vi "HOST.vi"() -> ()   [LabVIEW 2018]
uses:
  <vilib>/userdefined/High Color/nirio_resource_hc.ctl
  <instrlib>/niDCPower/nidcpower.llb/niDCPower Measurement Type.ctl
  <vilib>/FPGAPlugInAG/PXI-7953R/niLvFpga_Open_PXI-7953R.vi
  <vilib>/rvi/interface/common/dynamic/niFpgaDynamicAddResources.vi
  <vilib>/FPGAPlugInAG/Dynamic/niLvFpga_Reset_Dynamic.vi
  <vilib>/FPGAPlugInAG/Dynamic/niLvFpga_Run_Dynamic.vi
  <vilib>/Utility/error.llb/Error Cluster From Error Code.vi
  <vilib>/rvi/errors/niLvFpgaAdjustHostInterfaceError.vi
  <vilib>/FPGAPlugInAG/Dynamic/niLvFpga_Close_Dynamic.vi
  <vilib>/rvi/interface/nirviOpenFPGA/nirviOpenFPGA.xnode
  FPGA Bitfiles/GSENSE2020_FPGATarget_Target_dmqGfihq6bQ.lvbitx
  <vilib>/rvi/interface/nirviMethod/nirviMethod.xnode
  <vilib>/rvi/interface/nirviReadWriteControl/nirviReadWriteControl.xnode
  <vilib>/rvi/interface/nirviCloseFPGA/nirviCloseFPGA.xnode
  <vilib>/rvi/errors/niLvFpgaMergeErrorWithErrorCode.vi
  <vilib>/rvi/interface/Simulation/niFpgaSimulationCallBeginRW.vi
  <vilib>/FPGAPlugInAG/Dynamic/niLvFpga_ReadFifo_Dynamic.vi
  NiFpgaLv.dll
panel:
  in  "Коррекция":i32
  in  "SYNC":bool
  out "Temp":u16
  out "SEU":bool
  out "Записали адресов":u32
  out "SEU":u16
  out "REG":bool
  out "SEL":bool
  in  "Проверка \n   сбоев":bool
  in  "resource name 2":T1="PXI1Slot9"
  out "SPI_OUT":bool[](array[boolean])
  in  "W(T)/R(F)":bool=TRUE
  in  "Запись":bool[](array[boolean])=[TRUE, TRUE, FALSE, FALSE, FALSE, FALSE, FALSE, FALSE, TRUE, FALSE, TRUE, FALSE, TRUE, TRUE, TRUE, FALSE, FALSE, TRUE, FALSE, FALSE, TRUE, TRUE, FALSE, FALSE, TRUE, TRUE, FALSE, TRUE, TRUE, TRUE, FALSE, FALSE, FALSE, TRUE, TRUE, FALSE, FALSE, TRUE, TRUE, TRUE, TRUE, FALSE, FALSE, TRUE, FALSE, TRUE, FALSE, FALSE, FALSE, TRUE, FALSE, TRUE, TRUE, FALSE, TRUE, TRUE, TRUE, TRUE, TRUE, FALSE, TRUE, TRUE, TRUE, FALSE, TRUE, FALSE, FALSE, FALSE, TRUE, TRUE, TRUE, FALSE, FALSE, FALSE, FALSE, FALSE, FALSE, FALSE, FALSE, FALSE, FALSE, FALSE, FALSE, FALSE, FALSE, FALSE, TRUE, TRUE, TRUE, TRUE, FALSE, FALSE, FALSE, FALSE, FALSE, TRUE, TRUE, FALSE, TRUE, FALSE, TRUE, FALSE, FALSE, FALSE, FALSE, TRUE, FALSE, FALSE, FALSE, TRUE, TRUE, FALSE, TRUE, FALSE, FALSE, FALSE, TRUE, TRUE, TRUE, TRUE, TRUE, FALSE, FALSE, TRUE, FALSE, FALSE, FALSE, TRUE, TRUE, FALSE, TRUE, FALSE, FALSE, TRUE, TRUE, TRUE, TRUE, TRUE, TRUE, FALSE, FALSE, TRUE, TRUE, FALSE, FALSE, TRUE, TRUE, TRUE, TRUE, FALSE, FALSE, TRUE, TRUE, FALSE, FALSE, FALSE, FALSE, FALSE, TRUE, TRUE, FALSE, FALSE, TRUE, FALSE, FALSE, FALSE, FALSE, FALSE, FALSE, FALSE, FALSE, FALSE, FALSE, FALSE, FALSE, FALSE, FALSE, FALSE, FALSE, FALSE, TRUE, FALSE, FALSE, FALSE, FALSE, FALSE, FALSE, FALSE, TRUE, TRUE, FALSE, TRUE, TRUE, TRUE, TRUE, FALSE, TRUE, FALSE, FALSE, FALSE, FALSE, FALSE, FALSE, FALSE, FALSE, FALSE, FALSE, TRUE, TRUE, TRUE, TRUE, TRUE, TRUE, TRUE, TRUE, FALSE, FALSE, TRUE, TRUE, FALSE, FALSE, TRUE, TRUE, TRUE, TRUE, TRUE, TRUE, TRUE, FALSE, FALSE, FALSE, FALSE, TRUE, TRUE, TRUE, FALSE, TRUE, TRUE, FALSE, TRUE, FALSE, TRUE, FALSE, FALSE, FALSE, FALSE, FALSE, FALSE, FALSE, TRUE, TRUE, TRUE, FALSE, TRUE, TRUE, FALSE]
  in  "Top(T)/Bot(F)":bool=TRUE
  in  "SPI":bool
  in  "SEU":path=path "C:/VPL/LabView/GSENSE2020BSI/SEU"
  in  "Автомат":bool
  in  "SYS_RESET":bool
  in  "Хватит ждать!":bool
  in  "SEL_Time, ms":u32=100
  out "Номер образца":string="1"
  in  "Светлый (T)\nТемный (F)":bool
  in  "Frames":path=path "C:/VPL/LabView/GSENSE2020BSI/Frames"
  in  "ПРИМЕЧАНИЕ":string
  in  "SAVE":bool
  in  "122880":u32=122880
  in  "FRAME!":bool
  out "Картинка":bool
  out "Image":T2(plugin-control)
  out "Записали FIFO":bool
  in  "For FIFO (56)":i32=56
  in  "MOVIE":bool
  in  "SIM_SEL":bool
  out "VDD35":bool
  out "VDD20":bool
  out "3,3":bool
  out "LDC":bool
  out "VRH":bool
  in  "VDD35_selcur":dbl=0.25 caption="current limit" format="%_6p"
  in  "VDD20_selcur":dbl=0.4 caption="current limit" format="%_6p"
  in  "3,3_selcur":dbl=0.175 caption="current limit" format="%_6p"
  in  "LDC_selcur":dbl=0.01 caption="current limit" format="%_6p"
  in  "VRH_selcur":dbl=0.03 caption="current limit" format="%_6p"
  out "VDD35":u16
  out "VDD20":u16
  out "3,3":u16
  out "LDC":u16
  out "VRH":u16
  in  "Питание":bool
  in  "Стоп":bool
  in  "VDD35, V":dbl=3.51 caption="voltage level" format="%_6p"
  in  "3,3, V":dbl=3.3099999999999996 caption="voltage level" format="%_6p"
  in  "LDC, V":dbl=0.81 caption="voltage level" format="%_6p"
  in  "VRH, V":dbl=3.8099999999999996 caption="voltage level" format="%_6p"
  in  "VDD35_curlim":dbl=0.3 caption="current limit" format="%_6p"
  in  "VDD20_curlim":dbl=0.5 caption="current limit" format="%_6p"
  in  "3,3_curlim":dbl=0.2 caption="current limit" format="%_6p"
  in  "LDC_curlim":dbl=0.015 caption="current limit" format="%_6p"
  in  "LED_curlim":dbl=0.1 caption="current limit" format="%_6p"
  in  "VRH_curlim":dbl=0.05 caption="current limit" format="%_6p"
  out "VDD35_cur":dbl caption="measurement" format="%_6g"
  out "VDD20_cur":dbl caption="measurement" format="%_6g"
  out "3,3_cur":dbl caption="measurement" format="%_6g"
  out "LDC_cur":dbl caption="measurement" format="%_6g"
  out "LED_cur":dbl caption="measurement" format="%_6g"
  out "VRH_cur":dbl caption="measurement" format="%_6g"
  in  "VDD20, V":dbl=2.01 caption="voltage level" format="%_6p"
  in  "LED, V":dbl=6.0 caption="voltage level" format="%_6p"
  out "VDD35_char":dbl(graph)=-0.007753012065680951
  out "VDD20_char":dbl(graph)=6.909391540672134e-05
  out "3,3_char":dbl(graph)=9.424895165128459e-05
  out "LDC_char":dbl(graph)=-9.950040532110056e-06
  out "LED_char":dbl(graph)=9.067752968783287e-05
  out "VRH_char":dbl(graph)=1.5967060684808935e-06
  in  "LED":bool caption="output enabled"
  in  "0":refnum<k15>="PXI1Slot5" caption="1"
  in  "1":refnum<k15>="PXI1Slot6"
  in  "2":refnum<k15>="PXI1Slot7" caption="1"
  in  "SEL":path=path "C:/VPL/LabView/GSENSE2020BSI/SEL"
  out "Data":u8[][](array[numeric])
  out "Array":u32[][](array[numeric])
  # "Bot_ch - HIGH gain"
  # "Прибавка 124 сбоев связана с ТЭ"
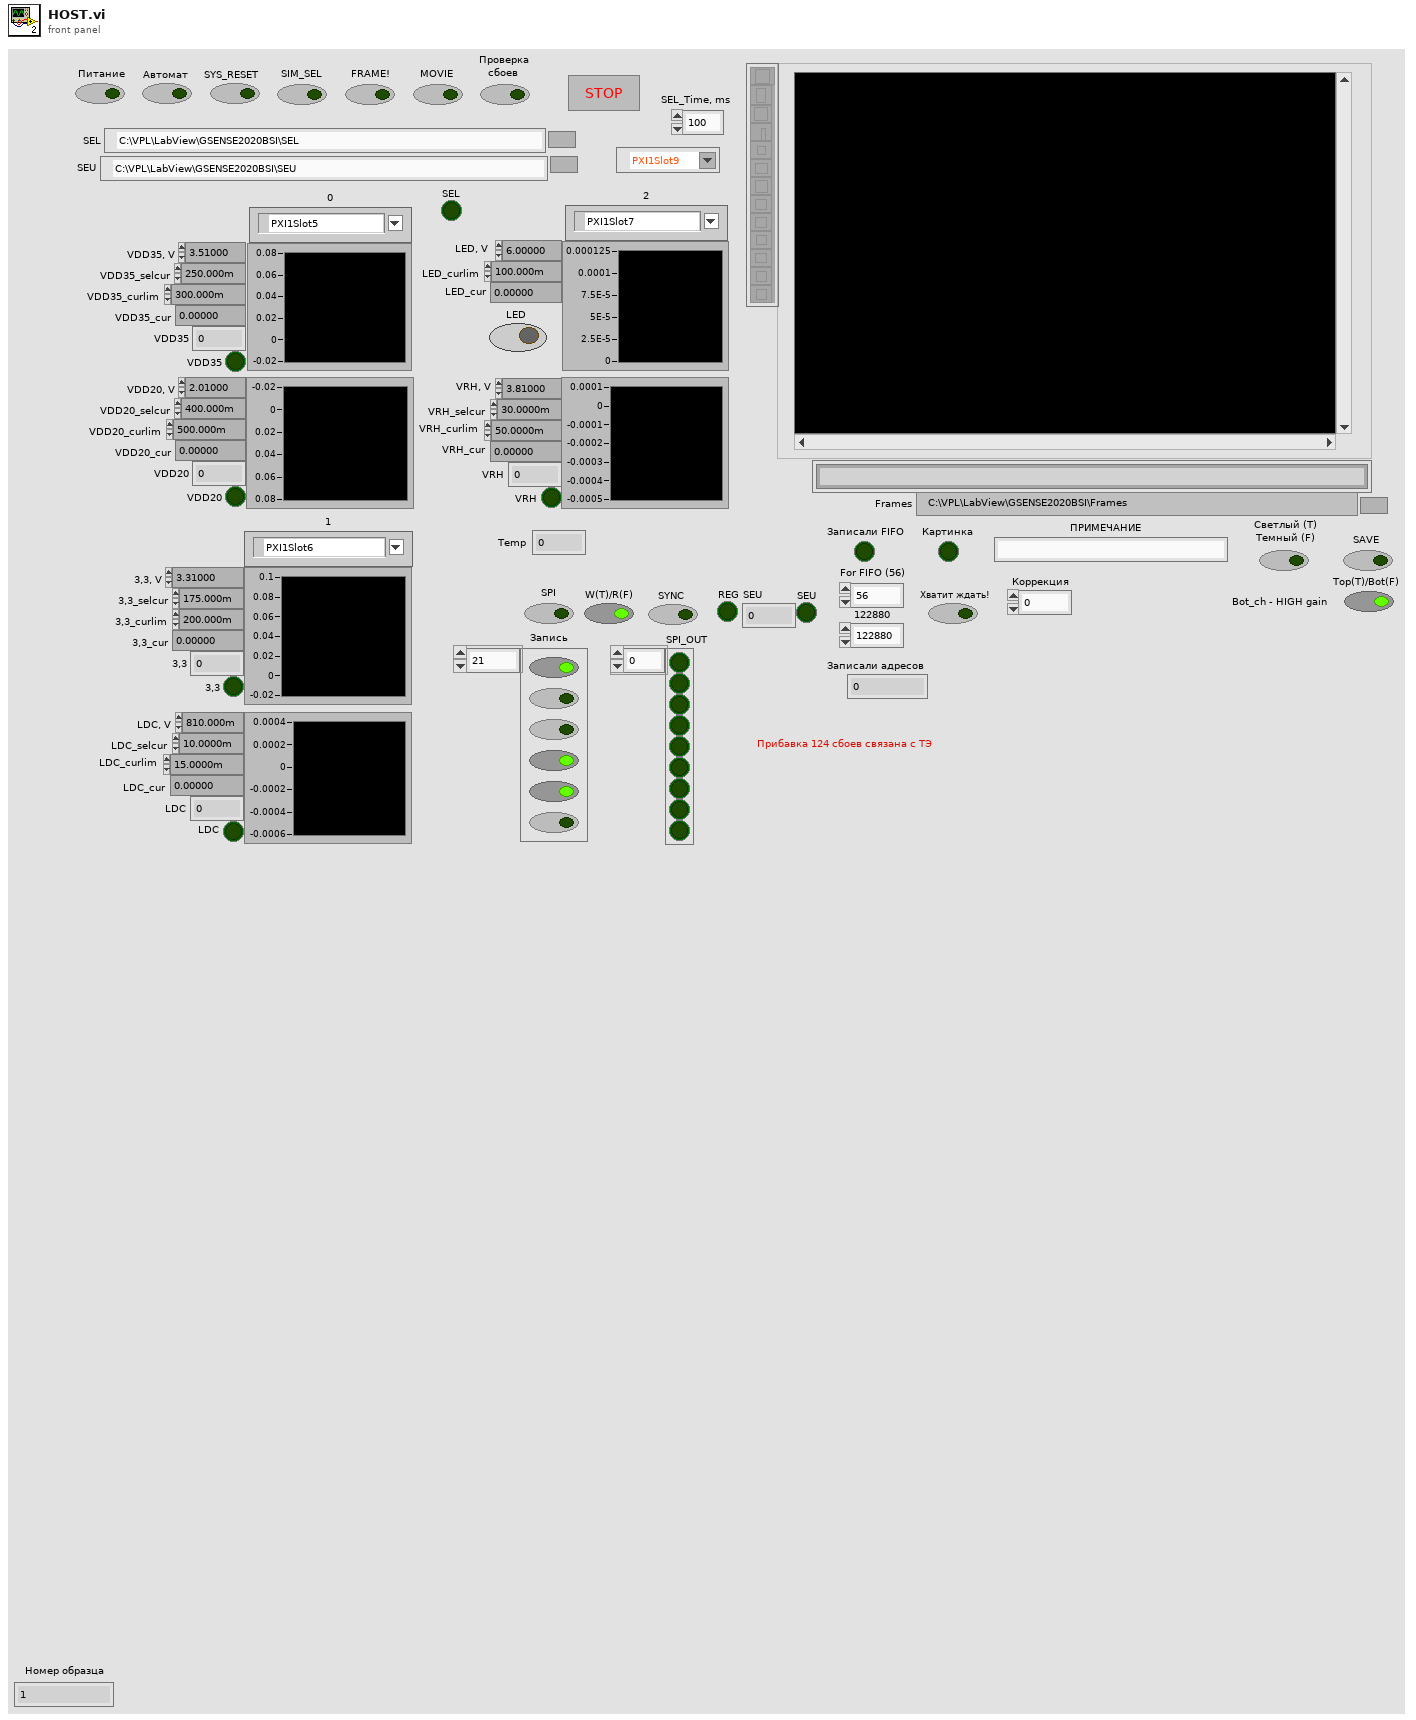
[diagram p1: front panel]
types:
  T1 = typedef "nirio_resource_hc.ctl" = tag
  T2 = typedef "IMAQ Image.ctl" = refnum<image>
  T3 = typedef "Image Type" = u32
  T4 = enum16{"open", "replace", "create", "open or create", "replace or create", "replace or create with confirmation"}
  T5 = typedef "niDCPower Measurement Type.ctl" = i32
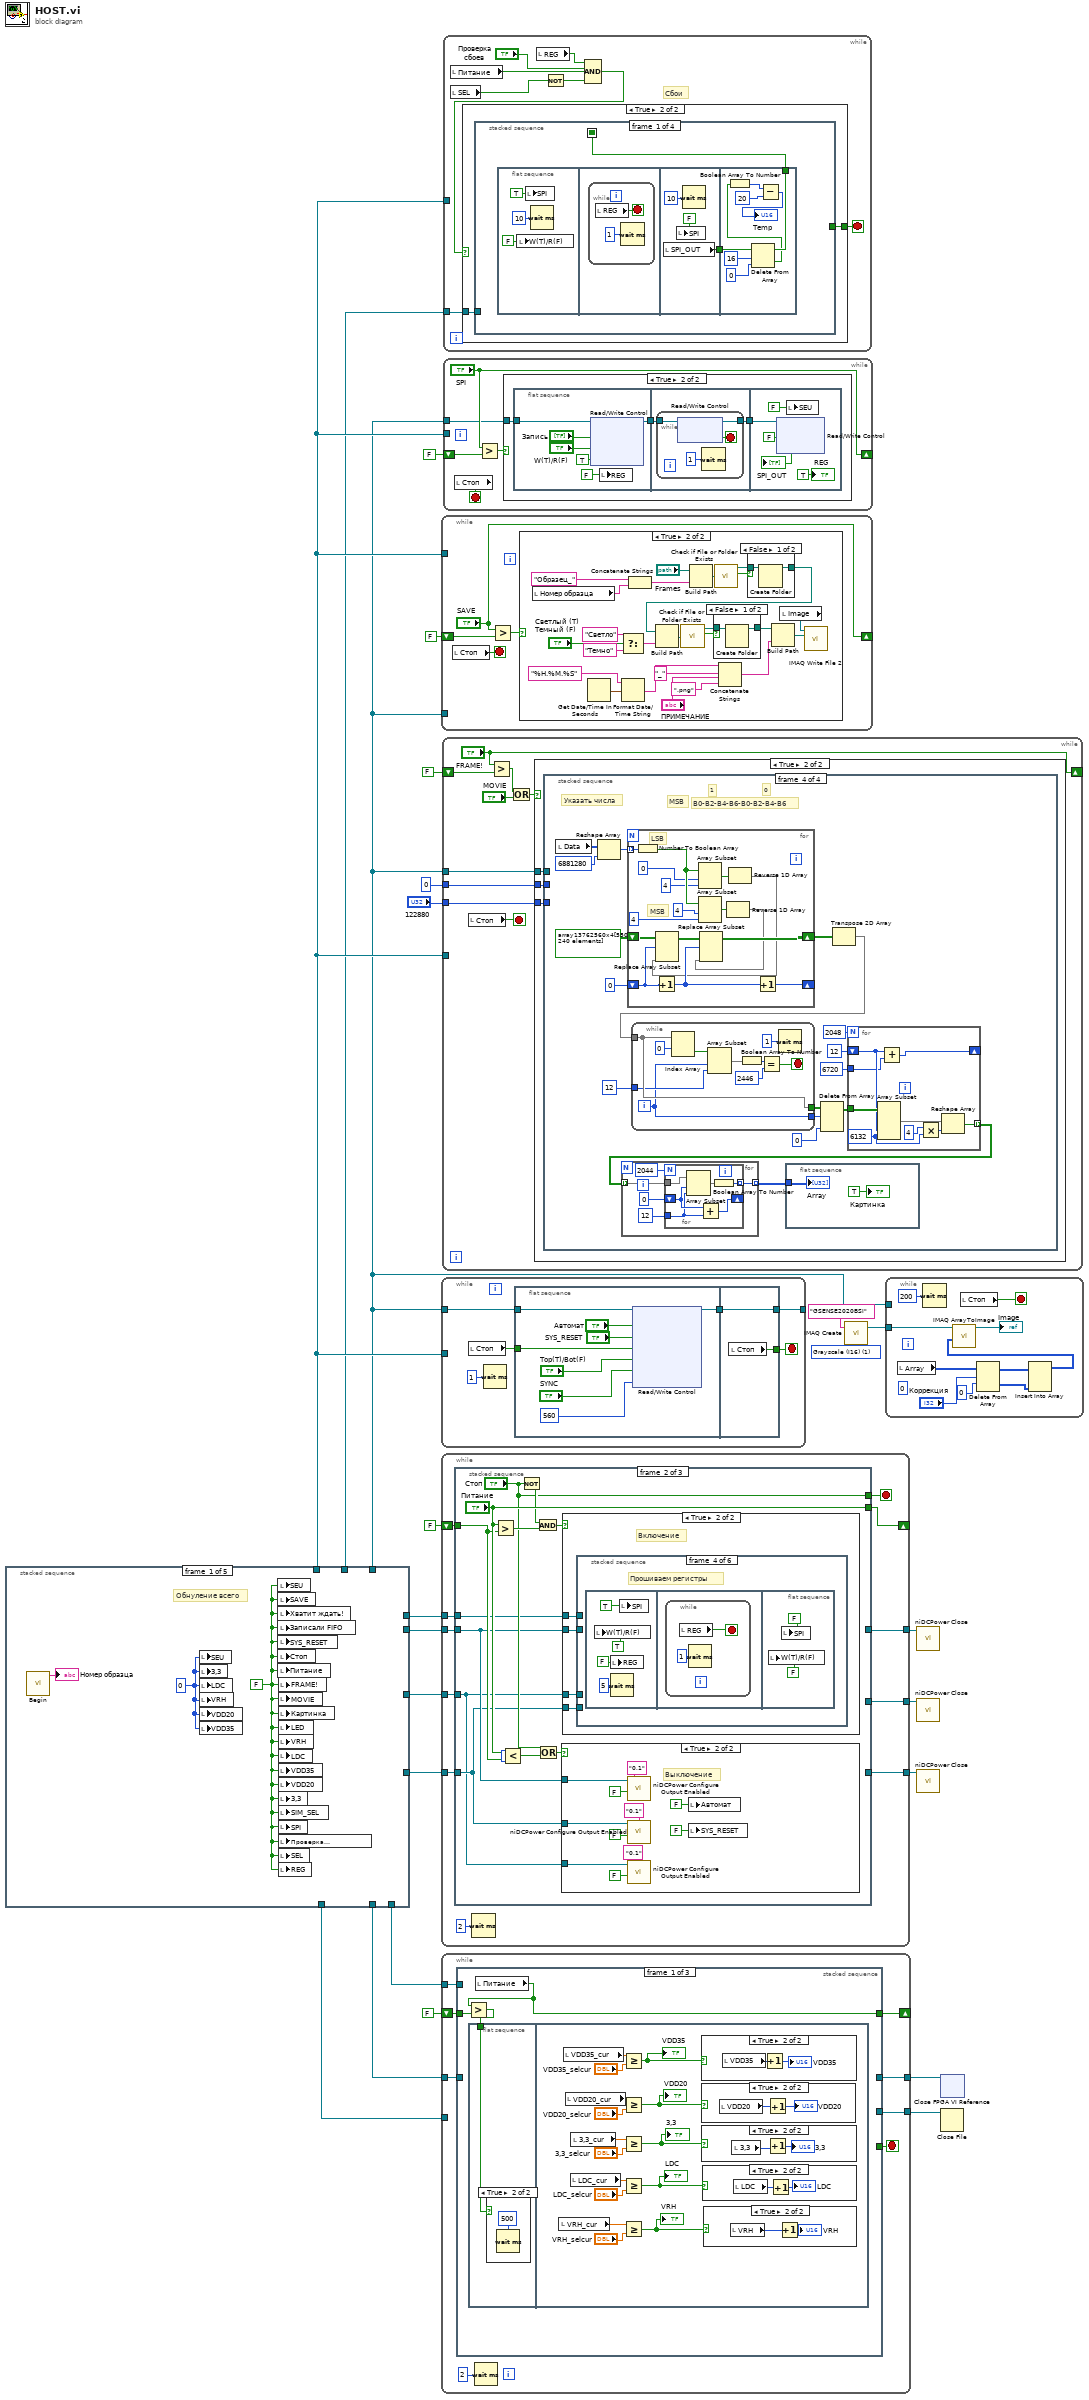
[diagram p0: block diagram]
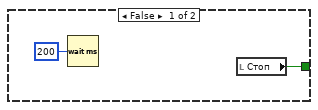
[diagram p2: hidden frame]
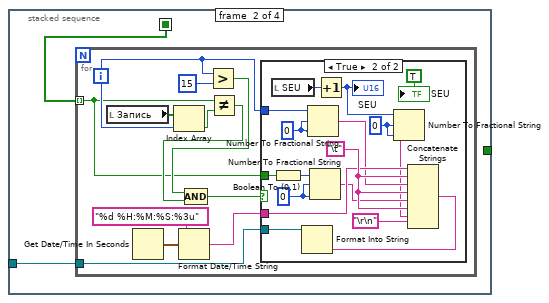
[diagram p3: hidden frame]
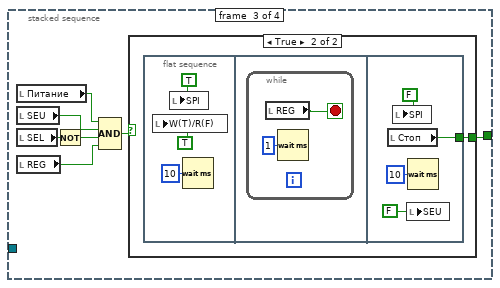
[diagram p5: hidden frame]
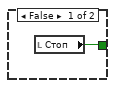
[diagram p6: hidden frame]
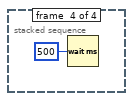
[diagram p7: hidden frame]
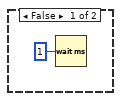
[diagram p8: hidden frame]
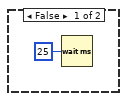
[diagram p9: hidden frame]
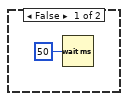
[diagram p12: hidden frame]
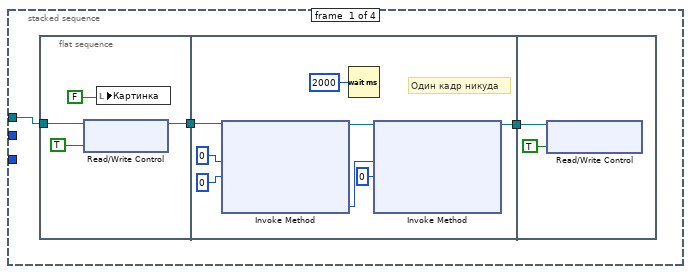
[diagram p13: hidden frame]
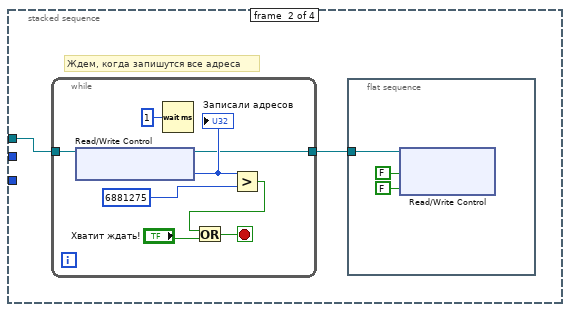
[diagram p14: hidden frame]
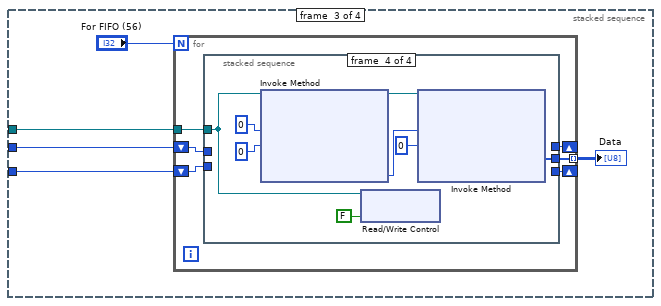
[diagram p15: hidden frame]
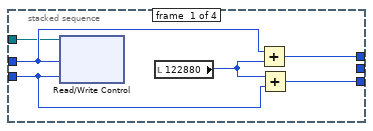
[diagram p16: hidden frame]
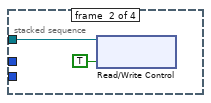
[diagram p17: hidden frame]
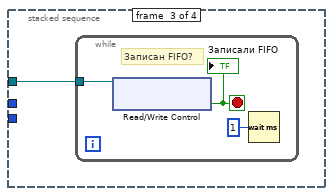
[diagram p18: hidden frame]
diagram:
  w3 = T3 1 items=["Grayscale (U8)", "Grayscale (I16)", "Grayscale (SGL)", "Complex (CSG)", "RGB (U32)", "HSL (U32)", "RGB (U64)"] ("Image Type")
  n1 = stacked-sequence {
    tunnel: [_ _ _ _ w103] -> w23
    tunnel: [_ _ _ _ w104] -> w25
    tunnel: [_ _ _ _ w108] -> w24
    tunnel: [_ _ _ w100 _] -> w1
    tunnel: [_ _ _ w100 _] -> w17
    tunnel: [_ w37 _ _ _] -> w18
    tunnel: [_ _ _ _ w104] -> w9
    tunnel: [_ _ _ _ w103] -> w12
    tunnel: [_ _ w67 _ _] -> w5
    tunnel: [_ _ _ w100 _] -> w6
    frame #0 {
      w26 = FALSE ("Стоп")
      w27 = u16 0 ("ADC")
      # "Обнуление всего"
      n2 = call "Begin.vi"() -> ("Номер образца 2"=→"Номер образца":string)  [unwired: 11 in]
      n3 = local write "SEU"(w27) -> ()
      n4 = local write "3,3"(w27) -> ()
      n5 = local write "LDC"(w27) -> ()
      n6 = local write "VRH"(w27) -> ()
      n7 = local write "VDD20"(w27) -> ()
      n8 = local write "VDD35"(w27) -> ()
      n9 = local write "SEU"(w26) -> ()
      n10 = local write "SAVE"(w26) -> ()
      n11 = local write "Хватит ждать!"(w26) -> ()
      n12 = local write "Записали FIFO"(w26) -> ()
      n13 = local write "SYS_RESET"(w26) -> ()
      n14 = local write "Стоп"(w26) -> ()
      n15 = local write "Питание"(w26) -> ()
      n16 = local write "FRAME!"(w26) -> ()
      n17 = local write "MOVIE"(w26) -> ()
      n18 = local write "Картинка"(w26) -> ()
      n19 = local write "LED"(w26) -> ()
      n20 = local write "VRH"(w26) -> ()
      n21 = local write "LDC"(w26) -> ()
      n22 = local write "VDD35"(w26) -> ()
      n23 = local write "VDD20"(w26) -> ()
      n24 = local write "3,3"(w26) -> ()
      n25 = local write "SIM_SEL"(w26) -> ()
      n26 = local write "SPI"(w26) -> ()
      n27 = local write "Проверка \n   сбоев"(w26) -> ()
      n28 = local write "SEL"(w26) -> ()
      n29 = local write "REG"(w26) -> ()
    }
    frame #1 {
      w31 = "\t"
      # "Лог по токам"
      n30 = local read "Номер образца"() -> (w59:string)
      n31 = Build Path(base path="SEL", name or relative path=w59) -> (appended path=w56:path)
      n32 = Get Date/Time In Seconds() -> (seconds since 1Jan1904=w53:timestamp)
      n33 = call <vilib>:"Check if File or Folder Exists.vi"("path"=w56) -> ("file or folder exists?"=w57:bool, "dup path"=w58:path)  [unwired: 8 in, 1 out]
      n34 = Format Date/Time String(time format string (%c)="%d %H.%M.%S", seconds (now)=w53) -> (date/time string=w51:string)  [unwired: 1 in]
      n35 = case shown="False" w57 {
        tunnel: w58 -> [w65 w66]
        tunnel: [w64 w66] -> w29
        frame False {
          n36 = Create Folder(path (use dialog)=w65) -> (created path=w64:path)  [unwired: 2 in, 2 out]
        }
        frame True {
        }
      }
      n37 = Concatenate Strings(w51, ".xls" ("string")) -> (w50:string)
      n38 = Build Path(base path=w29, name or relative path=w50) -> (appended path=w52:path)
      n39 = Open/Create/Replace File(file path (use dialog)=w52, operation (0:open)=T4."open or create", access (0:read/write)=enum16{"read/write", "read-only", "write-only"}."read/write") -> (refnum out=w54:refnum<file>)  [unwired: 3 in, 2 out]
      n40 = case shown="True" TRUE {
        tunnel: w54 -> [w60 w63]
        tunnel: [w60 w61] -> w49
        frame False {
        }
        frame True {
          n41 = Set File Position(refnum=w63, from (0:start)=enum16{"start", "end", "current"}."end") -> (refnum out=w61:refnum<file>)  [unwired: 2 in, 1 out]
        }
      }
      n42 = Format Into String(initial string=w49, "Time" ("input 1"), w31, "VDD35_cur", w31, "VDD20_cur", w31, "3,3_cur", w31, "LDC_cur", w31, "VRH_cur", w31, "VDD35_cur", w31, "VDD20_cur", w31, "3,3_cur", w31, "LDC_cur", w31, "VRH_cur", w31, "\r\n") -> (resulting string=w37:refnum<file>)  [unwired: 2 in, 1 out]
    }
    frame #2 {
      w70 = "\t"
      # "Лог по сбоям"
      n43 = local read "Номер образца"() -> (w74:string)
      n44 = Build Path(base path="SEU", name or relative path=w74) -> (appended path=w88:path)
      n45 = Get Date/Time In Seconds() -> (seconds since 1Jan1904=w86:timestamp)
      n46 = call <vilib>:"Check if File or Folder Exists.vi"("path"=w88) -> ("file or folder exists?"=w89:bool, "dup path"=w90:path)  [unwired: 8 in, 1 out]
      n47 = Format Date/Time String(time format string (%c)="%d %H.%M.%S", seconds (now)=w86) -> (date/time string=w84:string)  [unwired: 1 in]
      n48 = case shown="False" w89 {
        tunnel: w90 -> [w96 w97]
        tunnel: [w95 w97] -> w75
        frame False {
          n49 = Create Folder(path (use dialog)=w96) -> (created path=w95:path)  [unwired: 2 in, 2 out]
        }
        frame True {
        }
      }
      n50 = Concatenate Strings(w84, ".xls" ("string")) -> (w83:string)
      n51 = Build Path(base path=w75, name or relative path=w83) -> (appended path=w85:path)
      n52 = Open/Create/Replace File(file path (use dialog)=w85, operation (0:open)=T4."open or create", access (0:read/write)=enum16{"read/write", "read-only", "write-only"}."read/write") -> (refnum out=w87:refnum<file>)  [unwired: 3 in, 2 out]
      n53 = case shown="True" TRUE {
        tunnel: w87 -> [w91 w94]
        tunnel: [w91 w92] -> w82
        frame False {
        }
        frame True {
          n54 = Set File Position(refnum=w94, from (0:start)=enum16{"start", "end", "current"}."end") -> (refnum out=w92:refnum<file>)  [unwired: 2 in, 1 out]
        }
      }
      n55 = Format Into String(initial string=w82, "Time" ("input 1"), w70, "Регистр №" ("input 3"), w70, "Содержание" ("input 4"), w70, "Кол-во сбоев" ("input 7"), "\r\n") -> (resulting string=w67:refnum<file>)  [unwired: 2 in, 1 out]
    }
    frame #3 {
      n56 = xnode "Open FPGA VI Reference"("resource name"="resource name 2") -> ("FPGA VI Reference Out"=w98:refnum<k20>)  [unwired: 1 in, 1 out]
      n57 = xnode "Invoke Method"("FPGA VI Reference In"=w98) -> ("FPGA VI Reference Out"=w102:refnum<k20>, "error out"=w101:errorcluster)  [unwired: 1 in]
      n58 = xnode "Invoke Method"("FPGA VI Reference In"=w102, "error in"=w101) -> ("FPGA VI Reference Out"=w100:refnum<k20>)  [unwired: 1 in, 1 out]
    }
    frame #4 {
      # "Готово"
      n59 = call <instrlib>:"niDCPower Initialize.vi"("resource name"="2") -> ("error out"=w114:errorcluster, "instrument handle out"=w111:refnum<k15>)  [unwired: 3 in, 6 out]
      n60 = call <instrlib>:"niDCPower Initialize.vi"("resource name"="1") -> ("error out"=w112:errorcluster, "instrument handle out"=w109:refnum<k15>)  [unwired: 3 in, 6 out]
      n61 = call <instrlib>:"niDCPower Initialize.vi"("resource name"="0") -> ("error out"=w113:errorcluster, "instrument handle out"=w110:refnum<k15>)  [unwired: 3 in, 6 out]
      n62 = call <instrlib>:"niDCPower Configure Voltage Level.vi"("error in (no error)"=w114, "voltage level"=0.0, "channel name"="0,1", "instrument handle"=w111) -> ("instrument handle out"=w103:refnum<k15>)  [unwired: 6 in, 1 out]
      n63 = call <instrlib>:"niDCPower Configure Voltage Level.vi"("error in (no error)"=w112, "voltage level"=0.0, "channel name"="0,1", "instrument handle"=w109) -> ("instrument handle out"=w108:refnum<k15>)  [unwired: 6 in, 1 out]
      n64 = call <instrlib>:"niDCPower Configure Voltage Level.vi"("error in (no error)"=w113, "voltage level"=0.0, "channel name"="0,1", "instrument handle"=w110) -> ("instrument handle out"=w104:refnum<k15>)  [unwired: 6 in, 1 out]
    }
  }
  n65 = while {
    tunnel: w1 -> [w125]
    tunnel: [w124] -> _
    tunnel: w9 -> [_]
    stop <- w121 stop-if-true
    n66 = local read "Стоп"() -> (w123:bool)
    n67 = Wait (ms)(milliseconds to wait=u32 1) -> ()  [unwired: 1 out]
    n68 = flat-sequence {
      tunnel: w125 -> [w134]
      tunnel: w123 -> [w132]
      tunnel: [w133] -> w122
      tunnel: [w136] -> w124
      tunnel: w122 -> [w136]
      tunnel: [w135] -> w121
      frame #0 {
        n69 = xnode "Read/Write Control"("FPGA VI Reference In"=w134, "Автомат"="Автомат", "SYS_RESET"="SYS_RESET", "Стоп"=w132, "Top(T)/Bot(F)"="Top(T)/Bot(F)", "SYNC"="SYNC", "480"=u16 560) -> ("FPGA VI Reference Out"=w133:refnum<k20>)  [unwired: 1 in, 1 out]
      }
      frame #1 {
        n70 = local read "Стоп"() -> (w135:bool)
      }
    }
  }
  n71 = while {
    tunnel: w25 -> [w146]
    tunnel: w24 -> [w145]
    tunnel: w23 -> [w144]
    shift-right: [w141] -> _
    shift-left: FALSE -> [w142]
    tunnel: [w140] -> w21
    tunnel: [w139] -> w20
    tunnel: [w138] -> w19
    tunnel: w6 -> [w137]
    stop <- w143 stop-if-true
    n72 = stacked-sequence {
      tunnel: w144 -> [w158 w205 w256]
      tunnel: w146 -> [w160 w206 w258]
      tunnel: w145 -> [w159 w204 w257]
      tunnel: [_ "Стоп" _] -> w143
      tunnel: w142 -> [_ w213 _]
      tunnel: [_ "Питание" _] -> w141
      tunnel: [_ _ w258] -> w140
      tunnel: [_ _ w257] -> w139
      tunnel: [_ _ w256] -> w138
      tunnel: w137 -> [_ w203 _]
      frame #0 {
        w148 = T5 0 items=["Current", "Voltage"] ("measurement type")
        n73 = call <instrlib>:"niDCPower Configure Current Limit.vi"("current limit"="VDD35_curlim", "channel name"="0", "instrument handle"=w160) -> ("instrument handle out"=w183:refnum<k15>)  [unwired: 7 in, 1 out]
        n74 = call <instrlib>:"niDCPower Configure Current Limit.vi"("current limit"="VDD20_curlim", "channel name"="1", "instrument handle"=w160) -> ("instrument handle out"=w184:refnum<k15>)  [unwired: 7 in, 1 out]
        n75 = call <instrlib>:"niDCPower Configure Current Limit.vi"("current limit"="3,3_curlim", "channel name"="0", "instrument handle"=w159) -> ("instrument handle out"=w185:refnum<k15>)  [unwired: 7 in, 1 out]
        n76 = call <instrlib>:"niDCPower Configure Current Limit.vi"("current limit"="LDC_curlim", "channel name"="1", "instrument handle"=w159) -> ("instrument handle out"=w186:refnum<k15>)  [unwired: 7 in, 1 out]
        n77 = call <instrlib>:"niDCPower Configure Current Limit.vi"("current limit"="LED_curlim", "channel name"="0", "instrument handle"=w158) -> ("instrument handle out"=w187:refnum<k15>)  [unwired: 7 in, 1 out]
        n78 = call <instrlib>:"niDCPower Configure Current Limit.vi"("current limit"="VRH_curlim", "channel name"="1", "instrument handle"=w158) -> ("instrument handle out"=w188:refnum<k15>)  [unwired: 7 in, 1 out]
        n79 = call <instrlib>:"niDCPower Configure Voltage Level.vi"("voltage level"="VDD35, V", "channel name"="0", "instrument handle"=w183) -> ("instrument handle out"=w166:refnum<k15>)  [unwired: 7 in, 1 out]
        n80 = call <instrlib>:"niDCPower Configure Voltage Level.vi"("voltage level"="VDD20, V", "channel name"="1", "instrument handle"=w184) -> ("instrument handle out"=w165:refnum<k15>)  [unwired: 7 in, 1 out]
        n81 = call <instrlib>:"niDCPower Configure Voltage Level.vi"("voltage level"="3,3, V", "channel name"="0", "instrument handle"=w185) -> ("instrument handle out"=w164:refnum<k15>)  [unwired: 7 in, 1 out]
        n82 = call <instrlib>:"niDCPower Configure Voltage Level.vi"("voltage level"="LDC, V", "channel name"="1", "instrument handle"=w186) -> ("instrument handle out"=w163:refnum<k15>)  [unwired: 7 in, 1 out]
        n83 = call <instrlib>:"niDCPower Configure Voltage Level.vi"("voltage level"="LED, V", "channel name"="0", "instrument handle"=w187) -> ("instrument handle out"=w162:refnum<k15>)  [unwired: 7 in, 1 out]
        n84 = call <instrlib>:"niDCPower Configure Voltage Level.vi"("voltage level"="VRH, V", "channel name"="1", "instrument handle"=w188) -> ("instrument handle out"=w161:refnum<k15>)  [unwired: 7 in, 1 out]
        n85 = call <instrlib>:"niDCPower Measure.vi"("measurement type"=w148, "channel name"="0", "instrument handle"=w166) -> ("measurement"=→"VDD35_cur" →"VDD35_char":dbl)  [unwired: 6 in, 2 out]
        n86 = call <instrlib>:"niDCPower Measure.vi"("measurement type"=w148, "channel name"="1", "instrument handle"=w165) -> ("measurement"=→"VDD20_cur" →"VDD20_char":dbl)  [unwired: 6 in, 2 out]
        n87 = call <instrlib>:"niDCPower Measure.vi"("measurement type"=w148, "channel name"="0", "instrument handle"=w164) -> ("measurement"=→"3,3_cur" →"3,3_char":dbl)  [unwired: 6 in, 2 out]
        n88 = call <instrlib>:"niDCPower Measure.vi"("measurement type"=w148, "channel name"="1", "instrument handle"=w163) -> ("measurement"=→"LDC_cur" →"LDC_char":dbl)  [unwired: 6 in, 2 out]
        n89 = call <instrlib>:"niDCPower Measure.vi"("measurement type"=w148, "channel name"="0", "instrument handle"=w162) -> ("measurement"=→"LED_cur" →"LED_char":dbl, "instrument handle out"=w151:refnum<k15>)  [unwired: 6 in, 1 out]
        n90 = call <instrlib>:"niDCPower Measure.vi"("measurement type"=w148, "channel name"="1", "instrument handle"=w161) -> ("measurement"=→"VRH_cur" →"VRH_char":dbl)  [unwired: 6 in, 2 out]
        n91 = call <instrlib>:"niDCPower Configure Output Enabled.vi"("output enabled"="LED", "channel name"="0", "instrument handle"=w151) -> ()  [unwired: 7 in, 2 out]
      }
      frame #1 {
        n92 = Greater?(x="Питание", y=w213) -> (0:w210:bool)
        n93 = Less?(x="Питание", y=w213) -> (x < y?=w208:bool)
        n94 = Not(x="Стоп") -> (.not. x?=w209:bool)
        n95 = And(x=w209, y=w210) -> (x .and. y?=w212:bool)
        n96 = Or(x="Стоп", y=w208) -> (x .or. y?=w211:bool)
        n97 = case shown="True" w211 {
          tunnel: w206 -> [_ w225]
          tunnel: w205 -> [_ w224]
          tunnel: w204 -> [_ w223]
          frame False {
          }
          frame True {
            # "Выключение"
            n98 = call <instrlib>:"niDCPower Configure Output Enabled.vi"("output enabled"=FALSE, "channel name"="0,1", "instrument handle"=w225) -> ()  [unwired: 7 in, 2 out]
            n99 = call <instrlib>:"niDCPower Configure Output Enabled.vi"("output enabled"=FALSE, "channel name"="0,1", "instrument handle"=w224) -> ()  [unwired: 7 in, 2 out]
            n100 = call <instrlib>:"niDCPower Configure Output Enabled.vi"("output enabled"=FALSE, "channel name"="0,1", "instrument handle"=w223) -> ()  [unwired: 7 in, 2 out]
            n101 = local write "Автомат"(FALSE ("Автомат")) -> ()
            n102 = local write "SYS_RESET"(FALSE ("SYS_RESET")) -> ()
          }
        }
        n103 = case shown="True" w212 {
          tunnel: w206 -> [_ w229]
          tunnel: w204 -> [_ w228]
          tunnel: w205 -> [_ w227]
          tunnel: w203 -> [_ w226]
          frame False {
          }
          frame True {
            # "Включение"
            n104 = stacked-sequence {
              tunnel: w229 -> [w233 _ _ _ _ _]
              tunnel: w228 -> [w232 _ _ _ _ w251]
              tunnel: w227 -> [_ _ _ _ _ w250]
              tunnel: w226 -> [_ _ _ _ _ _]
              frame #0 {
                # "3,3"
                # "VDD20"
                # "VDD35(PIX)"
                n105 = call <instrlib>:"niDCPower Configure Output Enabled.vi"("output enabled"=TRUE, "channel name"="0", "instrument handle"=w233) -> ()  [unwired: 7 in, 2 out]
                n106 = call <instrlib>:"niDCPower Configure Output Enabled.vi"("output enabled"=TRUE, "channel name"="1", "instrument handle"=w233) -> ()  [unwired: 7 in, 2 out]
                n107 = call <instrlib>:"niDCPower Configure Output Enabled.vi"("output enabled"=TRUE, "channel name"="0", "instrument handle"=w232) -> ()  [unwired: 7 in, 2 out]
              }
              frame #1 {
                n108 = Wait (ms)(milliseconds to wait=u32 50) -> ()  [unwired: 1 out]
              }
              frame #2 {
                n109 = local write "Автомат"(TRUE ("Автомат")) -> ()
              }
              frame #3 {
                # "Прошиваем регистры"
                n110 = flat-sequence {
                  frame #0 {
                    n111 = local write "W(T)/R(F)"(TRUE ("W(T)/R(F)")) -> ()
                    n112 = local write "REG"(FALSE ("REG")) -> ()
                    n113 = Wait (ms)(milliseconds to wait=u32 5) -> ()  [unwired: 1 out]
                    n114 = local write "SPI"(TRUE ("SPI")) -> ()
                  }
                  frame #1 {
                    n115 = while {
                      stop <- w244 stop-if-true
                      n116 = local read "REG"() -> (w244:bool)
                      n117 = Wait (ms)(milliseconds to wait=u32 1) -> ()  [unwired: 1 out]
                    }
                  }
                  frame #2 {
                    n118 = local write "W(T)/R(F)"(FALSE ("W(T)/R(F)")) -> ()
                    n119 = local write "SPI"(FALSE ("SPI")) -> ()
                  }
                }
              }
              frame #4 {
                n120 = Wait (ms)(milliseconds to wait=u32 1) -> ()  [unwired: 1 out]
              }
              frame #5 {
                # "VRH"
                # "LDC"
                n121 = call <instrlib>:"niDCPower Configure Output Enabled.vi"("output enabled"=TRUE, "channel name"="1", "instrument handle"=w251) -> ()  [unwired: 7 in, 2 out]
                n122 = call <instrlib>:"niDCPower Configure Output Enabled.vi"("output enabled"=TRUE, "channel name"="1", "instrument handle"=w250) -> ()  [unwired: 7 in, 2 out]
                n123 = local write "SYS_RESET"(TRUE ("SYS_RESET")) -> ()
              }
            }
          }
        }
      }
      frame #2 {
      }
    }
    n124 = Wait (ms)(milliseconds to wait=u32 2) -> ()  [unwired: 1 out]
  }
  n125 = while {
    tunnel: w17 -> [w261]
    shift-right: [w265] -> _
    shift-left: FALSE ("Питание") -> [w266]
    tunnel: w18 -> [w263]
    tunnel: w12 -> [_]
    tunnel: [w260] -> w11
    tunnel: [w259] -> w10
    stop <- w262 stop-if-true
    n126 = stacked-sequence {
      tunnel: w266 -> [w269 _ _]
      tunnel: [w268 _ _] -> w265
      tunnel: w263 -> [_ w330 _]
      tunnel: [_ _ w346] -> w262
      tunnel: w261 -> [_ _ w345]
      tunnel: [_ w297 _] -> w260
      tunnel: [_ _ w336] -> w259
      frame #0 {
        n127 = flat-sequence {
          tunnel: w267 -> [w270]
          frame #0 {
            n128 = case shown="True" w270 {
              frame False {
              }
              frame True {
                n129 = Wait (ms)(milliseconds to wait=u32 500) -> ()  [unwired: 1 out]
              }
            }
          }
          frame #1 {
            n130 = local read "VRH_cur"() -> (w277:dbl)
            n131 = local read "VDD35_cur"() -> (w279:dbl)
            n132 = local read "VDD20_cur"() -> (w280:dbl)
            n133 = local read "LDC_cur"() -> (w282:dbl)
            n134 = local read "3,3_cur"() -> (w281:dbl)
            n135 = Greater Or Equal?(x=w279, y="VDD35_selcur") -> (x >= y?=w276:bool)
            "VDD35" <- w276
            n136 = Greater Or Equal?(x=w280, y="VDD20_selcur") -> (x >= y?=w275:bool)
            "VDD20" <- w275
            n137 = Greater Or Equal?(x=w281, y="3,3_selcur") -> (x >= y?=w274:bool)
            "3,3" <- w274
            n138 = Greater Or Equal?(x=w282, y="LDC_selcur") -> (x >= y?=w273:bool)
            "LDC" <- w273
            n139 = Greater Or Equal?(x=w277, y="VRH_selcur") -> (x >= y?=w272:bool)
            "VRH" <- w272
            n140 = case shown="True" w276 {
              frame False {
              }
              frame True {
                n141 = local read "VDD35"() -> (w295:u16)
                n142 = Increment(x=w295) -> (x+1=→"VDD35":u16)
              }
            }
            n143 = case shown="True" w275 {
              frame False {
              }
              frame True {
                n144 = local read "VDD20"() -> (w293:u16)
                n145 = Increment(x=w293) -> (x+1=→"VDD20":u16)
              }
            }
            n146 = case shown="True" w274 {
              frame False {
              }
              frame True {
                n147 = local read "3,3"() -> (w291:u16)
                n148 = Increment(x=w291) -> (x+1=→"3,3":u16)
              }
            }
            n149 = case shown="True" w273 {
              frame False {
              }
              frame True {
                n150 = local read "LDC"() -> (w289:u16)
                n151 = Increment(x=w289) -> (x+1=→"LDC":u16)
              }
            }
            n152 = case shown="True" w272 {
              frame False {
              }
              frame True {
                n153 = local read "VRH"() -> (w287:u16)
                n154 = Increment(x=w287) -> (x+1=→"VRH":u16)
              }
            }
          }
        }
        n155 = local read "Питание"() -> (w268:bool)
        n156 = Greater?(x=w268, y=w269) -> (0:w267:bool)
      }
      frame #1 {
        w312 = "\t"
        w328 = i16 0 ("width (-)")
        w329 = i16 3 ("width (-)")
        n157 = local read "VDD35_cur"() -> (w327:dbl)
        n158 = local read "VDD20_cur"() -> (w326:dbl)
        n159 = Get Date/Time In Seconds() -> (seconds since 1Jan1904=w335:timestamp)
        n160 = local read "VRH_cur"() -> (w301:dbl)
        n161 = local read "LDC_cur"() -> (w302:dbl)
        n162 = local read "3,3_cur"() -> (w303:dbl)
        n163 = local read "VDD35"() -> (w325:u16)
        n164 = local read "VDD20"() -> (w324:u16)
        n165 = local read "VDD35"() -> (w311:bool)
        n166 = local read "VDD20"() -> (w310:bool)
        n167 = local read "VRH"() -> (w298:u16)
        n168 = local read "VRH"() -> (w304:bool)
        n169 = local read "LDC"() -> (w299:u16)
        n170 = local read "LDC"() -> (w308:bool)
        n171 = local read "3,3"() -> (w300:u16)
        n172 = local read "3,3"() -> (w309:bool)
        n173 = Format Date/Time String(time format string (%c)="%d %H:%M:%S:%3u", seconds (now)=w335) -> (date/time string=w323:string)  [unwired: 1 in]
        n174 = Compound Arithmetic op=OR(w311, w310, w309, w308, w304) -> (w307:bool)
        n175 = Number To Fractional String(number=w327, width (-)=w329, precision (6)=w329) -> (F-format string=w322:string)  [unwired: 1 in]
        n176 = Number To Fractional String(number=w326, width (-)=w329, precision (6)=w329) -> (F-format string=w321:string)  [unwired: 1 in]
        n177 = Number To Fractional String(number=w303, width (-)=w329, precision (6)=w329) -> (F-format string=w320:string)  [unwired: 1 in]
        n178 = Number To Fractional String(number=w302, width (-)=w329, precision (6)=w329) -> (F-format string=w319:string)  [unwired: 1 in]
        n179 = Number To Fractional String(number=w301, width (-)=w329, precision (6)=w329) -> (F-format string=w318:string)  [unwired: 1 in]
        n180 = Number To Fractional String(number=w325, width (-)=w328, precision (6)=w328) -> (F-format string=w317:string)  [unwired: 1 in]
        n181 = Number To Fractional String(number=w324, width (-)=w328, precision (6)=w328) -> (F-format string=w316:string)  [unwired: 1 in]
        n182 = Number To Fractional String(number=w300, width (-)=w328, precision (6)=w328) -> (F-format string=w315:string)  [unwired: 1 in]
        n183 = Number To Fractional String(number=w299, width (-)=w328, precision (6)=w328) -> (F-format string=w314:string)  [unwired: 1 in]
        n184 = Number To Fractional String(number=w298, width (-)=w328, precision (6)=w328) -> (F-format string=w313:string)  [unwired: 1 in]
        n185 = Select(t="!!!", s=w307, f="") -> (s? t:f=w306:string)
        n186 = Concatenate Strings(w323, w312, w322, w312, w321, w312, w320, w312, w319, w312, w318, w312, w317, w312, w316, w312, w315, w312, w314, w312, w313, w312, w306, "\r\n") -> (w331:string)
        n187 = Format Into String(initial string=w330, w331) -> (resulting string=w297:refnum<file>)  [unwired: 2 in, 1 out]
      }
      frame #2 {
        n188 = local read "VDD35"() -> (w344:bool)
        n189 = local read "VDD20"() -> (w343:bool)
        n190 = local read "VRH"() -> (w337:bool)
        n191 = local read "LDC"() -> (w341:bool)
        n192 = local read "3,3"() -> (w342:bool)
        n193 = local read "Питание"() -> (w338:bool)
        n194 = Compound Arithmetic op=OR(w344, w343, w342, w341, w337, "SIM_SEL") -> (w339:bool)
        "SEL" <- w339
        n195 = case shown="True" w339 {
          tunnel: [w348 w356] -> w346
          tunnel: w345 -> [w347 w355]
          tunnel: w338 -> [_ w352]
          tunnel: [w347 w351] -> w336
          frame False {
            n196 = local read "Стоп"() -> (w348:bool)
          }
          frame True {
            n197 = flat-sequence {
              tunnel: w355 -> [w360]
              tunnel: [w358] -> w353
              tunnel: w352 -> [w358]
              tunnel: [w357] -> w349
              tunnel: [w363] -> w354
              tunnel: w353 -> [w363]
              tunnel: [w362] -> w350
              tunnel: w349 -> [w362]
              tunnel: [w367] -> w356
              tunnel: w354 -> [w366]
              tunnel: [w365] -> w351
              tunnel: w350 -> [w365]
              frame #0 {
                n198 = local write "Питание"(FALSE ("Питание")) -> ()
                n199 = xnode "Read/Write Control"("FPGA VI Reference In"=w360, "Автомат"=FALSE ("Линейки")) -> ("FPGA VI Reference Out"=w357:refnum<k20>)  [unwired: 1 in, 1 out]
              }
              frame #1 {
                n200 = Wait (ms)(milliseconds to wait="SEL_Time, ms") -> ()  [unwired: 1 out]
              }
              frame #2 {
                n201 = local write "Питание"(w366) -> ()
                n202 = local read "Стоп"() -> (w367:bool)
              }
            }
          }
        }
      }
    }
    n203 = Wait (ms)(milliseconds to wait=u32 2) -> ()  [unwired: 1 out]
  }
  n204 = while {
    shift-right: ["SAVE"] -> _
    shift-left: FALSE ("SAVE") -> [w370]
    tunnel: w1 -> [_]
    tunnel: w9 -> [_]
    stop <- w371 stop-if-true
    n205 = local read "Стоп"() -> (w371:bool)
    n206 = Greater?(x="SAVE", y=w370) -> (0:w369:bool)
    n207 = case shown="True" w369 {
      frame False {
        n208 = Wait (ms)(milliseconds to wait=u32 25) -> ()  [unwired: 1 out]
      }
      frame True {
        n209 = local read "Номер образца"() -> (w378:string)
        n210 = Get Date/Time In Seconds() -> (seconds since 1Jan1904=w392:timestamp)
        n211 = Select(t="Светло", s="Светлый (T)\nТемный (F)", f="Темно") -> (s? t:f=w393:string)
        n212 = Format Date/Time String(time format string (%c)="%H.%M.%S", seconds (now)=w392) -> (date/time string=w396:string)  [unwired: 1 in]
        n213 = Concatenate Strings("Образец_" ("string"), w378) -> (w376:string)
        n214 = Build Path(base path="Frames", name or relative path=w376) -> (appended path=w387:path)
        n215 = call <vilib>:"Check if File or Folder Exists.vi"("path"=w387) -> ("file or folder exists?"=w386:bool, "dup path"=w385:path)  [unwired: 8 in, 1 out]
        n216 = Concatenate Strings(w396, "_", "ПРИМЕЧАНИЕ", ".png" ("element")) -> (w395:string)
        n217 = case shown="False" w386 {
          tunnel: w385 -> [w402 w403]
          tunnel: [w401 w403] -> w375
          frame False {
            n218 = Create Folder(path (use dialog)=w402) -> (created path=w401:path)  [unwired: 2 in, 2 out]
          }
          frame True {
          }
        }
        n219 = Build Path(base path=w375, name or relative path=w393) -> (appended path=w388:path)
        n220 = call <vilib>:"Check if File or Folder Exists.vi"("path"=w388) -> ("file or folder exists?"=w389:bool, "dup path"=w390:path)  [unwired: 8 in, 1 out]
        n221 = case shown="False" w389 {
          tunnel: w390 -> [w399 w400]
          tunnel: [w398 w400] -> w394
          frame False {
            n222 = Create Folder(path (use dialog)=w399) -> (created path=w398:path)  [unwired: 2 in, 2 out]
          }
          frame True {
          }
        }
        n223 = Build Path(base path=w394, name or relative path=w395) -> (appended path=w391:path)
        n224 = local read "Image"() -> (w379:T2)
        n225 = call-poly "IMAQ Write File 2"("File Path"=w391, "Image"=w379) -> ()  [unwired: 8 in, 2 out]
      }
    }
  }
  n226 = while {
    tunnel: w1 -> [w409]
    shift-right: ["FRAME!"] -> _
    shift-left: FALSE ("FRAME!") -> [w411]
    tunnel: u32 0 -> [w408]
    tunnel: "122880" -> [w407]
    tunnel: w9 -> [_]
    stop <- w412 stop-if-true
    n227 = local read "Стоп"() -> (w412:bool)
    n228 = Greater?(x="FRAME!", y=w411) -> (0:w405:bool)
    n229 = Or(x=w405, y="MOVIE") -> (x .or. y?=w406:bool)
    n230 = case shown="True" w406 {
      tunnel: w409 -> [_ w416]
      tunnel: w408 -> [_ w415]
      tunnel: w407 -> [_ w414]
      frame False {
        n231 = Wait (ms)(milliseconds to wait=u32 50) -> ()  [unwired: 1 out]
      }
      frame True {
        n232 = stacked-sequence {
          tunnel: w416 -> [w419 w435 w451 _]
          tunnel: w415 -> [_ _ w450 _]
          tunnel: w414 -> [_ _ w449 _]
          frame #0 {
            n233 = flat-sequence {
              tunnel: w419 -> [w422]
              tunnel: [w423] -> w418
              tunnel: w418 -> [w426]
              tunnel: [w425] -> w417
              tunnel: w417 -> [w432]
              frame #0 {
                n234 = xnode "Read/Write Control"("FPGA VI Reference In"=w422, "Управление"=TRUE ("Кадр в память")) -> ("FPGA VI Reference Out"=w423:refnum<k20>)  [unwired: 1 in, 1 out]
                n235 = local write "Картинка"(FALSE ("Картинка")) -> ()
              }
              frame #1 {
                # "Один кадр никуда"
                n236 = xnode "Invoke Method"("FPGA VI Reference In"=w426, "Number of Elements"=u32 0, "Timeout (ms)"=0) -> ("FPGA VI Reference Out"=w431:refnum<k20>, "Elements Remaining"=w430:u32)  [unwired: 1 in, 2 out]
                n237 = Wait (ms)(milliseconds to wait=u32 2000) -> ()  [unwired: 1 out]
                n238 = xnode "Invoke Method"("FPGA VI Reference In"=w431, "Number of Elements"=w430, "Timeout (ms)"=0) -> ("FPGA VI Reference Out"=w425:refnum<k20>)  [unwired: 1 in, 3 out]
              }
              frame #2 {
                n239 = xnode "Read/Write Control"("FPGA VI Reference In"=w432, "Кадр в память"=TRUE) -> ()  [unwired: 1 in, 2 out]
              }
            }
          }
          frame #1 {
            # "Ждем, когда запишутся все адреса"
            n240 = while {
              tunnel: w435 -> [w444]
              tunnel: [w439] -> w434
              stop <- w446 stop-if-true
              n241 = xnode "Read/Write Control"("FPGA VI Reference In"=w444) -> ("FPGA VI Reference Out"=w439:refnum<k20>, "Записали адресов"=w443:u32)  [unwired: 1 in, 1 out]
              "Записали адресов" <- w443
              n242 = Wait (ms)(milliseconds to wait=u32 1) -> ()  [unwired: 1 out]
              n243 = Greater?(x=w443, y=u32 6881275) -> (0:w441:bool)
              n244 = Or(x=w441, y="Хватит ждать!") -> (x .or. y?=w446:bool)
            }
            n245 = flat-sequence {
              tunnel: w434 -> [w437]
              frame #0 {
                n246 = xnode "Read/Write Control"("FPGA VI Reference In"=w437, "Управление"=FALSE, "Кадр в память"=FALSE) -> ()  [unwired: 1 in, 2 out]
              }
            }
          }
          frame #2 {
            n247 = for {
              N: "For FIFO (56)" -> [_]
              shift-right: [w455] -> _
              shift-left: w450 -> [w457]
              shift-right: [w454] -> _
              shift-left: w449 -> [w456]
              tunnel: w451 -> [w453]
              tunnel: [w452] -> w447 mode=indexing
              n248 = stacked-sequence {
                tunnel: [_ _ _ w475] -> w452
                tunnel: [w463 _ _ _] -> w455
                tunnel: [w462 _ _ _] -> w454
                tunnel: w457 -> [w460 _ _ _]
                tunnel: w456 -> [w461 _ _ _]
                tunnel: w453 -> [w459 w464 w466 w470]
                frame #0 {
                  n249 = xnode "Read/Write Control"("FPGA VI Reference In"=w459, "Нач_адр"=w460, "Кон_адр"=w461) -> ()  [unwired: 1 in, 2 out]
                  n250 = local read "122880"() -> (w458:u32)
                  n251 = Add(x=w460, y=w458) -> (x+y=w463:u32)
                  n252 = Add(x=w458, y=w461) -> (x+y=w462:u32)
                }
                frame #1 {
                  n253 = xnode "Read/Write Control"("FPGA VI Reference In"=w464, "Кадр на ПК"=TRUE ("HOST")) -> ()  [unwired: 1 in, 2 out]
                }
                frame #2 {
                  n254 = while {
                    tunnel: w466 -> [w467]
                    stop <- w469 stop-if-true
                    # "Записан FIFO?"
                    n255 = xnode "Read/Write Control"("FPGA VI Reference In"=w467) -> ("Записали FIFO"=w469:bool)  [unwired: 1 in, 2 out]
                    "Записали FIFO" <- w469
                    n256 = Wait (ms)(milliseconds to wait=u32 1) -> ()  [unwired: 1 out]
                  }
                }
                frame #3 {
                  n257 = xnode "Invoke Method"("FPGA VI Reference In"=w470, "Number of Elements"=u32 0, "Timeout (ms)"=0) -> ("FPGA VI Reference Out"=w476:refnum<k20>, "Elements Remaining"=w477:u32)  [unwired: 1 in, 2 out]
                  n258 = xnode "Read/Write Control"("FPGA VI Reference In"=w470, "Кадр на ПК"=FALSE ("HOST")) -> ()  [unwired: 1 in, 2 out]
                  n259 = xnode "Invoke Method"("FPGA VI Reference In"=w476, "Number of Elements"=w477, "Timeout (ms)"=0) -> ("Data"=w475:u8[])  [unwired: 1 in, 3 out]
                }
              }
            }
            "Data" <- w447
          }
          frame #3 {
            # "Указать числа"
            # "0"
            # "MSB"
            # "1"
            # "B0-B2-B4-B6-B0-B2-B4-B6"
            n260 = local read "Data"() -> (w494:u8[][])
            n261 = Reshape Array(w494, 6881280 ("Requested Number of Elements")) -> (w492:u8[])
            n262 = for {
              tunnel: w492 -> [w536] mode=indexing
              shift-right: [w537] -> w488
              shift-left: bool[][] array13762560x4[55050240 elements] -> [w542]
              shift-right: [w539] -> _
              shift-left: 0 -> [w541]
              # "LSB"
              # "MSB"
              n263 = Number To Boolean Array(number=w536) -> (Boolean array=w535:bool[])
              n264 = Increment(x=w541) -> (x+1=w540:i32)
              n265 = Array Subset(array=w535, index=0 ("length"), length=4 ("index")) -> (w530:bool[])
              n266 = Array Subset(array=w535, index=4 ("length"), length=4 ("index")) -> (w528:bool[])
              n267 = Reverse 1D Array(array=w528) -> (reversed array=w527:bool[])
              n268 = Reverse 1D Array(array=w530) -> (reversed array=w529:bool[])
              n269 = Replace Array Subset(array=w542, new element=w529, index (row)=w541) -> (w538:bool[][])  [unwired: 1 in]
              n270 = Replace Array Subset(array=w538, new element=w527, index (row)=w540) -> (w537:bool[][])  [unwired: 1 in]
              n271 = Increment(x=w540) -> (x+1=w539:i32)
            }
            n272 = flat-sequence {
              tunnel: w478 -> [w496]
              frame #0 {
                "Array" <- w496
                "Картинка" <- TRUE
              }
            }
            n273 = Transpose 2D Array(2D array=w488) -> (transposed array=w487:bool[][])
            n274 = while {
              tunnel: w487 -> [w523]
              tunnel: 12 -> [w520]
              tunnel: [w523] -> w486
              tunnel: [w517] -> w484
              i -> [w517]
              stop <- w518 stop-if-true
              n275 = Index Array(array=w523, index (row)=0) -> (element=w521:bool[])  [unwired: 1 in]
              n276 = Array Subset(array=w521, index=w517, length=w520) -> (w519:bool[])
              n277 = Boolean Array To Number(Boolean array=w519) -> (number=w526:u32)
              n278 = Equal?(x=w526, y=u32 2446) -> (x = y?=w518:bool)
              n279 = Wait (ms)(milliseconds to wait=u32 1) -> ()  [unwired: 1 out]
            }
            n280 = Delete From Array(array=w486, length=w484, index (col)=0 ("disabled index (col)")) -> (array with subset deleted=w483:bool[][])  [unwired: 1 in, 1 out]
            n281 = for {
              N: 2048 -> [_]
              tunnel: w483 -> [w516]
              tunnel: 6720 -> [w511]
              shift-right: [w514] -> _
              shift-left: 12 -> [w513]
              tunnel: [w512] -> w479 mode=indexing
              w509 = 6132 ("length")
              n282 = Array Subset(array=w516, index (col)=w513, length (col)=w509) -> (w515:bool[][])  [unwired: 2 in]
              n283 = Add(x=w513, y=w511) -> (x+y=w514:i32)
              n284 = Multiply(x=4, y=w509) -> (x*y=w510:i32)
              n285 = Reshape Array(w515, w510) -> (w512:bool[])
            }
            n286 = for {
              tunnel: w479 -> [w501] mode=indexing
              tunnel: [w497] -> w478 mode=indexing
              n287 = for {
                N: 2044 -> [_]
                tunnel: w501 -> [w502]
                tunnel: [w506] -> w497 mode=indexing
                tunnel: 12 -> [w504]
                shift-right: [w503] -> _
                shift-left: 0 -> [w505]
                n288 = Array Subset(array=w502, index=w505, length=w504) -> (w507:bool[])
                n289 = Add(x=w505, y=w504) -> (x+y=w503:i32)
                n290 = Boolean Array To Number(Boolean array=w507) -> (number=w506:u32)
              }
            }
          }
        }
      }
    }
  }
  n291 = while {
    tunnel: w9 -> [_]
    tunnel: w5 -> [w549]
    stop <- w550 stop-if-true
    # "Сбои"
    n292 = local read "Питание"() -> (w546:bool)
    n293 = local read "SEL"() -> (w545:bool)
    n294 = local read "REG"() -> (w548:bool)
    n295 = Not(x=w545) -> (.not. x?=w544:bool)
    n296 = Compound Arithmetic op=AND(w548, "Проверка \n   сбоев", w546, w544) -> (w543:bool)
    n297 = case shown="True" w543 {
      tunnel: [w551 w554] -> w550
      tunnel: w549 -> [_ w553]
      frame False {
        n298 = Wait (ms)(milliseconds to wait=u32 200) -> ()  [unwired: 1 out]
        n299 = local read "Стоп"() -> (w551:bool)
      }
      frame True {
        n300 = stacked-sequence {
          seq-local: [w555 _ _ _] -> [_ w573 _ _]
          tunnel: [_ _ w610 _] -> w554
          tunnel: w553 -> [_ w574 _ _]
          frame #0 {
            n301 = flat-sequence {
              tunnel: [w562] -> w556
              tunnel: w556 -> [w570]
              tunnel: [w569] -> w555
              frame #0 {
                n302 = local write "W(T)/R(F)"(FALSE ("W(T)/R(F)")) -> ()
                n303 = local write "SPI"(TRUE ("SPI")) -> ()
                n304 = Wait (ms)(milliseconds to wait=u32 10) -> ()  [unwired: 1 out]
              }
              frame #1 {
                n305 = while {
                  stop <- w561 stop-if-true
                  n306 = local read "REG"() -> (w561:bool)
                  n307 = Wait (ms)(milliseconds to wait=u32 1) -> ()  [unwired: 1 out]
                }
              }
              frame #2 {
                n308 = local read "SPI_OUT"() -> (w562:bool[])
                n309 = local write "SPI"(FALSE ("SPI")) -> ()
                n310 = Wait (ms)(milliseconds to wait=u32 10) -> ()  [unwired: 1 out]
              }
              frame #3 {
                n311 = Delete From Array(array=w570, length=16, index=0) -> (deleted portion=w568:bool[], array with subset deleted=w569:bool[])
                n312 = Boolean Array To Number(Boolean array=w568) -> (number=w566:u16)
                n313 = Subtract(x=w566, y=u16 20) -> (x-y=→"Temp":u16)
              }
            }
          }
          frame #1 {
            n314 = for {
              tunnel: w573 -> [w576] mode=indexing
              tunnel: w574 -> [w575]
              i -> [w581]
              n315 = local read "Запись"() -> (w586:bool[])
              n316 = Get Date/Time In Seconds() -> (seconds since 1Jan1904=w584:timestamp)
              n317 = Index Array(array=w586, index=w581) -> (element=w585:bool)
              n318 = Format Date/Time String(time format string (%c)="%d %H:%M:%S:%3u", seconds (now)=w584) -> (date/time string=w582:string)  [unwired: 1 in]
              n319 = Greater?(x=w581, y=15) -> (0:w579:bool)
              n320 = Not Equal?(x=w576, y=w585) -> (x != y?=w578:bool)
              n321 = Compound Arithmetic op=AND(w579, w578) -> (w577:bool)
              n322 = case shown="True" w577 {
                tunnel: w581 -> [_ w603]
                tunnel: w582 -> [_ w597]
                tunnel: w576 -> [_ w589]
                tunnel: w575 -> [_ w588]
                frame False {
                }
                frame True {
                  w591 = i16 0 ("width (-)")
                  w598 = i16 0 ("width (-)")
                  w600 = "\t"
                  w602 = i16 0 ("width (-)")
                  n323 = local read "SEU"() -> (w594:u16)
                  n324 = Boolean To (0,1)(Boolean=w589) -> (0, 1=w599:i16)
                  n325 = Number To Fractional String(number=w603, width (-)=w602, precision (6)=w602) -> (F-format string=w596:string)  [unwired: 1 in]
                  n326 = Number To Fractional String(number=w599, width (-)=w598, precision (6)=w598) -> (F-format string=w595:string)  [unwired: 1 in]
                  n327 = Increment(x=w594) -> (x+1=w592:u16)
                  "SEU" <- w592
                  n328 = Number To Fractional String(number=w592, width (-)=w591, precision (6)=w591) -> (F-format string=w593:string)  [unwired: 1 in]
                  n329 = Concatenate Strings(w597, w600, w596, w600, w595, w600, w593, "\r\n") -> (w587:string)
                  n330 = Format Into String(initial string=w588, w587) -> ()  [unwired: 2 in, 2 out]
                  "SEU" <- TRUE ("SEU")
                }
              }
            }
          }
          frame #2 {
            n331 = local read "Питание"() -> (w608:bool)
            n332 = local read "SEU"() -> (w607:bool)
            n333 = local read "SEL"() -> (w605:bool)
            n334 = local read "REG"() -> (w604:bool)
            n335 = Not(x=w605) -> (.not. x?=w606:bool)
            n336 = Compound Arithmetic op=AND(w608, w607, w606, w604) -> (w609:bool)
            n337 = case shown="True" w609 {
              tunnel: [w611 w612] -> w610
              frame False {
                n338 = local read "Стоп"() -> (w611:bool)
              }
              frame True {
                n339 = flat-sequence {
                  tunnel: [w620] -> w612
                  frame #0 {
                    n340 = local write "W(T)/R(F)"(TRUE ("W(T)/R(F)")) -> ()
                    n341 = local write "SPI"(TRUE ("SPI")) -> ()
                    n342 = Wait (ms)(milliseconds to wait=u32 10) -> ()  [unwired: 1 out]
                  }
                  frame #1 {
                    n343 = while {
                      stop <- w616 stop-if-true
                      n344 = local read "REG"() -> (w616:bool)
                      n345 = Wait (ms)(milliseconds to wait=u32 1) -> ()  [unwired: 1 out]
                    }
                  }
                  frame #2 {
                    n346 = local read "Стоп"() -> (w620:bool)
                    n347 = local write "SPI"(FALSE ("SPI")) -> ()
                    n348 = local write "SEU"(FALSE ("SEU")) -> ()
                    n349 = Wait (ms)(milliseconds to wait=u32 10) -> ()  [unwired: 1 out]
                  }
                }
              }
            }
          }
          frame #3 {
            n350 = Wait (ms)(milliseconds to wait=u32 500) -> ()  [unwired: 1 out]
          }
        }
      }
    }
  }
  n351 = while {
    tunnel: w9 -> [_]
    tunnel: w1 -> [w623]
    shift-right: ["SPI"] -> _
    shift-left: FALSE ("SPI") -> [w625]
    stop <- w627 stop-if-true
    n352 = local read "Стоп"() -> (w627:bool)
    n353 = Greater?(x="SPI", y=w625) -> (0:w624:bool)
    n354 = case shown="True" w624 {
      tunnel: w623 -> [_ w631]
      frame False {
        n355 = Wait (ms)(milliseconds to wait=u32 1) -> ()  [unwired: 1 out]
      }
      frame True {
        n356 = flat-sequence {
          tunnel: w631 -> [w637]
          tunnel: [w634] -> w630
          tunnel: w630 -> [w639]
          tunnel: [w638] -> w629
          tunnel: w629 -> [w648]
          frame #0 {
            n357 = xnode "Read/Write Control"("FPGA VI Reference In"=w637, "SPI_IN"="Запись", "W(T)/R(F)"="W(T)/R(F)", "SPI"=TRUE) -> ("FPGA VI Reference Out"=w634:refnum<k20>)  [unwired: 1 in, 1 out]
            n358 = local write "REG"(FALSE ("REG")) -> ()
          }
          frame #1 {
            n359 = while {
              tunnel: w639 -> [w643]
              tunnel: [w640] -> w638
              stop <- w642 stop-if-true
              n360 = xnode "Read/Write Control"("FPGA VI Reference In"=w643) -> ("FPGA VI Reference Out"=w640:refnum<k20>, "SPI_OFF"=w642:bool)  [unwired: 1 in, 1 out]
              n361 = Wait (ms)(milliseconds to wait=u32 1) -> ()  [unwired: 1 out]
            }
          }
          frame #2 {
            n362 = xnode "Read/Write Control"("FPGA VI Reference In"=w648, "SPI"=FALSE) -> ("SPI_OUT"=→"SPI_OUT":bool[])  [unwired: 1 in, 2 out]
            n363 = local write "SEU"(FALSE ("SEU")) -> ()
            "REG" <- TRUE ("REG")
          }
        }
      }
    }
  }
  n364 = call "IMAQ Create"("Image Name"="GSENSE2020BSI", "Image Type"=w3) -> ("New Image"=w2:T2)  [unwired: 3 in, 1 out]
  n365 = while {
    tunnel: w2 -> [w656]
    tunnel: w1 -> [_]
    stop <- w649 stop-if-true
    (unwired) 0 ("index")
    n366 = local read "Array"() -> (w654:u32[][])
    n367 = Wait (ms)(milliseconds to wait=u32 200) -> ()  [unwired: 1 out]
    n368 = local read "Стоп"() -> (w649:bool)
    n369 = Delete From Array(array=w654, length="Коррекция", index (row)=0) -> (deleted portion=w651:u32[][], array with subset deleted=w655:u32[][])  [unwired: 1 in]
    n370 = Insert Into Array(array=w655, new element=w651) -> (w650:u32[][])  [unwired: 2 in]
    n371 = call "IMAQ ArrayToImage"("Image Pixels (I16)"=w650, "Image"=w656) -> ("Image Out"=→"Image":T2)  [unwired: 8 in, 1 out]
  }
  n372 = call <instrlib>:"niDCPower Close.vi"("instrument handle"=w21) -> ()  [unwired: 10 in, 1 out]
  n373 = call <instrlib>:"niDCPower Close.vi"("instrument handle"=w20) -> ()  [unwired: 10 in, 1 out]
  n374 = call <instrlib>:"niDCPower Close.vi"("instrument handle"=w19) -> ()  [unwired: 10 in, 1 out]
  n375 = Close File(refnum=w11) -> ()  [unwired: 1 in, 2 out]
  n376 = xnode "Close FPGA VI Reference"("FPGA VI Reference In"=w10) -> ()  [unwired: 1 in, 1 out]
